vi "Refresh Channel Names and Defaults.vi"(8 "error in (no error)":errorcluster, 10 "engine configuration in":refnum<class "engine configuration.lvclass">, 11 "SHM configuration in":refnum<class "Shared Memory configuration.lvclass">) -> (0 "error out":errorcluster, 2 "engine configuration out":refnum<class "engine configuration.lvclass">, 3 "SHM configuration out":refnum<class "Shared Memory configuration.lvclass">)   [LabVIEW 2014, in "Shared Memory editor node.lvclass"]
uses:
  Shared Memory editor node.lvclass
  <vilib>/NI/Module Execution Interface/Engine Configuration/engine configuration.lvclass
  module/configuration/Shared Memory configuration.lvclass
  <vilib>/NI/Configuration Framework/serializable configuration/NISE_CEF_serializable configuration.lvclass/NISE_CEF_serializable configuration.ctl
  module/configuration/Shared Memory configuration.lvclass/Shared Memory configuration.ctl
  <vilib>/NI/Tag Bus/tag/tag descriptor.lvclass/tag descriptor.ctl
  <vilib>/Utility/LVClass/Get LV Class Name.vi
  <vilib>/NI/Configuration Framework/error generator/NISE_error generator.vi
  <vilib>/NI/Tag Bus Module Framework/channel/TBM channel.lvclass
  <vilib>/NI/Tag Bus/tag/tag descriptor.lvclass
  <vilib>/NI/Configuration Framework/serializable configuration/NISE_CEF_serializable configuration.lvclass
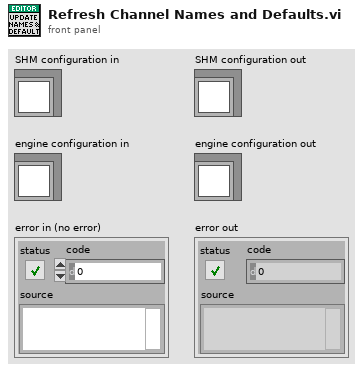
[diagram p1: front panel]
types:
  T1 = typedef "Shared Memory configuration.lvclass/Line.ctl" = cluster{"channel":refnum<class "TBM channel.lvclass">}
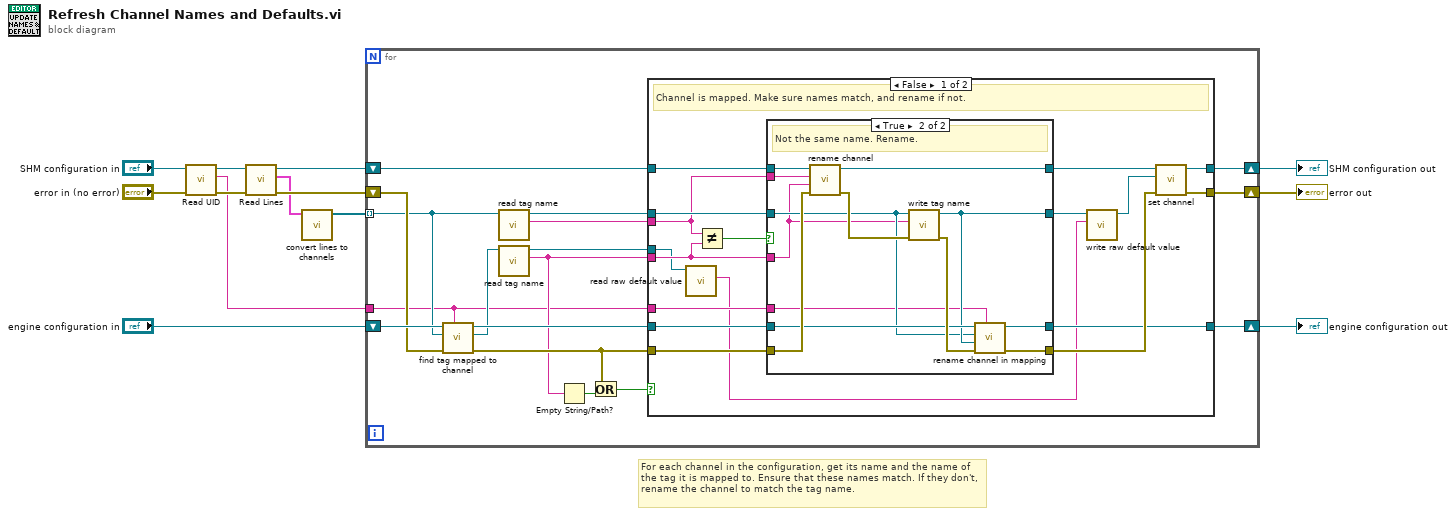
[diagram p0: block diagram]
diagram:
  # "For each channel in the configuration, get its name and the name of the tag it is mapped to. Ensure that these names match. If they don't, rename the channel to match the tag name."
  n1 = call <vilib>:"Read UID.vi"("error in"="error in (no error)", "configuration in"="SHM configuration in") -> ("error out"=w6:errorcluster, "instance id"=w1:string, "configuration out"=w7:refnum<class "Shared Memory configuration.lvclass">)  [unwired: 7 in]
  n2 = call "Read Lines.vi"("error in"=w6, "Shared Memory configuration in"=w7) -> ("error out"=w4:errorcluster, "Lines"=w2:T1[], "Shared Memory configuration out"=w5:refnum<class "Shared Memory configuration.lvclass">)  [unwired: 7 in]
  n3 = call "convert lines to channels.vi"("Lines in"=w2) -> ("channels out"=w3:refnum<class "TBM channel.lvclass">[])  [unwired: 9 in, 1 out]
  n4 = for {
    tunnel: w3 -> [w20] mode=indexing
    shift-right: [w25] -> w10
    shift-left: w4 -> [w26]
    shift-right: [w24] -> w12
    shift-left: w5 -> [w28]
    shift-right: [w23] -> w11
    shift-left: "engine configuration in" -> [w30]
    tunnel: w1 -> [w14]
    n5 = call <vilib>:"find tag mapped to channel.vi"("owner"=w14, "error in"=w26, "channel"=w20, "engine configuration in"=w30) -> ("error out"=w17:errorcluster, "tag"=w22:refnum<class "tag descriptor.lvclass">, "engine configuration out"=w27:refnum<class "engine configuration.lvclass">)  [unwired: 5 in]
    n6 = call <vilib>:"read tag name.vi"("system tag in"=w20) -> ("name"=w18:string, "system tag out"=w19:refnum<class "TBM channel.lvclass">)  [unwired: 8 in, 1 out]
    n7 = call <vilib>:"read tag name.vi"("system tag in"=w22) -> ("name"=w15:string, "system tag out"=w21:refnum<class "tag descriptor.lvclass">)  [unwired: 8 in, 1 out]
    n8 = Empty String/Path?(string/path=w15) -> (empty?=w16:bool)
    n9 = Or(x=w17, y=w16) -> (x .or. y?=w29:bool)
    n10 = case shown="False" w29 {
      tunnel: w21 -> [w33 _]
      tunnel: w15 -> [w34 _]
      tunnel: w18 -> [w35 _]
      tunnel: w19 -> [w46 _]
      tunnel: w28 -> [w47 w66]
      tunnel: w27 -> [w39 w67]
      tunnel: w17 -> [w36 w65]
      tunnel: [w42 w65] -> w25
      tunnel: [w41 w66] -> w24
      tunnel: [w37 w67] -> w23
      tunnel: w14 -> [w32 _]
      frame False {
        # "Channel is mapped. Make sure names match, and rename if not."
        n11 = call <vilib>:"read raw default value.vi"("system tag in"=w33) -> ("raw default"=w31:string)  [unwired: 8 in, 2 out]
        n12 = Not Equal?(x=w35, y=w34) -> (x != y?=w40:bool)
        n13 = case shown="True" w40 {
          tunnel: w47 -> [w51 w63]
          tunnel: w35 -> [_ w62]
          tunnel: w46 -> [w49 w54]
          tunnel: w34 -> [_ w53]
          tunnel: w39 -> [w50 w56]
          tunnel: [w51 w61] -> w44
          tunnel: [w50 w60] -> w37
          tunnel: [w48 w59] -> w38
          tunnel: w36 -> [w48 w58]
          tunnel: [w49 w55] -> w45
          tunnel: w32 -> [_ w52]
          frame False {
            # "Same name. Nothing to do."
          }
          frame True {
            # "Not the same name. Rename."
            n14 = call "rename channel.vi"("error in"=w58, "new name"=w53, "old name"=w62, "SHM configuration in"=w63) -> ("error out"=w64:errorcluster, "SHM configuration out"=w61:refnum<class "Shared Memory configuration.lvclass">)  [unwired: 6 in]
            n15 = call <vilib>:"write tag name.vi"("error in"=w64, "name"=w53, "system tag in"=w54) -> ("error out"=w57:errorcluster, "system tag out"=w55:refnum<class "TBM channel.lvclass">)  [unwired: 7 in]
            n16 = call <vilib>:"rename channel in mapping.vi"("owner ID"=w52, "error in"=w57, "new channel"=w55, "old channel"=w54, "engine configuration in"=w56) -> ("error out"=w59:errorcluster, "engine configuration out"=w60:refnum<class "engine configuration.lvclass">)  [unwired: 5 in]
          }
        }
        n17 = call <vilib>:"write raw default value.vi"("raw default"=w31, "system tag in"=w45) -> ("system tag out"=w43:refnum<class "TBM channel.lvclass">)  [unwired: 8 in, 1 out]
        n18 = call "set channel.vi"("error in"=w38, "TBM channel in"=w43, "SHM configuration in"=w44) -> ("error out"=w42:errorcluster, "SHM configuration out"=w41:refnum<class "Shared Memory configuration.lvclass">)  [unwired: 7 in]
      }
      frame True {
        # "Channel not mapped to tag. Nothing to do."
      }
    }
  }
  "engine configuration out" <- w11
  "SHM configuration out" <- w12
  "error out" <- w10
